vi "Lookup Config Value.vi"(8 "error in (no error)":errorcluster, 10 "Config Key":string, 11 "Device in":refnum<class "Device.lvclass">) -> (0 "error out":errorcluster, 1 "Found?":bool, 2 "Value":string, 3 "Device out":refnum<class "Device.lvclass">)   [LabVIEW 2020, in "HAL.lvlib" / "Device.lvclass"]
doc: "Concrete device classes can pull configuration values as strings using this VI. It is up to the concrete device class to convert the string value to the correct data type."
uses:
  Device.lvclass
  Device.lvclass/Device.ctl
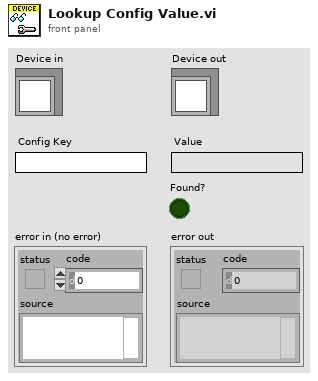
[diagram p1: front panel]
types:
  T1 = typedef "HAL.lvlib/Device.lvclass/Ref Data.ctl" = cluster{"Config Keys":string[], "Config Values":string[], "Cal Expires":timestamp, "Name":string, "Comment":string, "State":T2, "Error":errorcluster}
  T2 = typedef "HAL.lvlib/Device.lvclass/Device State.ctl" = enum16{"Uninitialized", "Initialized", "Ready", "Running", "Error"}
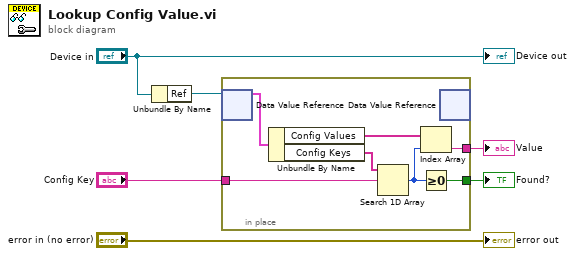
[diagram p0: block diagram]
diagram:
  n1 = Unbundle By Name("Device in") -> ("Ref"=w5:refnum<data-value>)
  n2 = in-place {
    in-place-border: "Config Key" -> [w11]
    in-place-border: [w9] -> w2
    in-place-border: [w7] -> w1
    n3 = in-place-dvr #1(w5) -> (w13:T1)  [unwired: 1 out]
    n4 = Unbundle By Name(w13) -> ("Config Values"=w10:string[], "Config Keys"=w12:string[])
    n5 = Search 1D Array(1D array=w12, element=w11) -> (index of element=w8:i32)  [unwired: 1 in]
    n6 = Index Array(array=w10, index=w8) -> (element=w9:string)
    n7 = Greater Or Equal To 0?(x=w8) -> (x >= 0?=w7:bool)
    n8 = in-place-dvr #1() -> ()  [unwired: 1 in, 2 out]
  }
  "Value" <- w2
  "Found?" <- w1
  "error out" <- "error in (no error)"
  "Device out" <- "Device in"
